vi "Close.vi"(0 "Application Ref":refnum<vi>, 5 "VI Reference":refnum<vi>, 11 "error in":errorcluster) -> (15 "error out":errorcluster)   [LabVIEW 2016, in "Drona.lvlib"]
doc: "Closes the given application and VI reference"
uses:
  Drona.lvlib
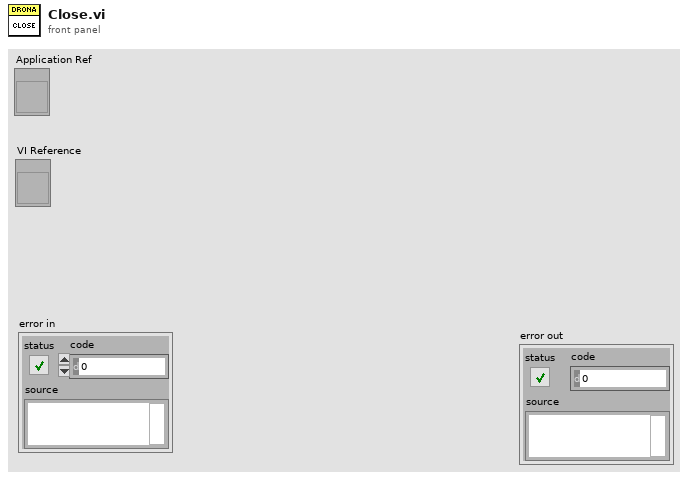
[diagram p1: front panel]
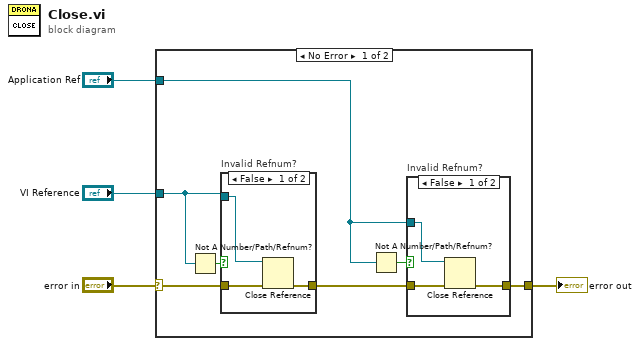
[diagram p0: block diagram]
diagram:
  n1 = case shown="No Error" "error in" {
    selector: "error in" -> [w5 w20]
    tunnel: [w10 w20] -> w4
    tunnel: "VI Reference" -> [w9 _]
    tunnel: "Application Ref" -> [w7 _]
    frame No Error {
      n2 = Not A Number/Path/Refnum?(number/path/refnum=w9) -> (NaN/Path/Refnum?=w8:bool)
      n3 = case "Invalid Refnum?" shown="False" w8 {
        tunnel: w5 -> [w18 w19]
        tunnel: [w17 w19] -> w11
        tunnel: w9 -> [w16 _]
        frame False {
          n4 = Close Reference(reference=w16, error in (no error)=w18) -> (error out=w17:errorcluster)
        }
        frame True {
        }
      }
      n5 = Not A Number/Path/Refnum?(number/path/refnum=w7) -> (NaN/Path/Refnum?=w6:bool)
      n6 = case "Invalid Refnum?" shown="False" w6 {
        tunnel: w11 -> [w14 w15]
        tunnel: [w13 w15] -> w10
        tunnel: w7 -> [w12 _]
        frame False {
          n7 = Close Reference(reference=w12, error in (no error)=w14) -> (error out=w13:errorcluster)
        }
        frame True {
        }
      }
    }
    frame Error {
    }
  }
  "error out" <- w4
